vi "VIH HelpGen - Control Label to Control ID.vi"(11 "Control Name":string) -> (3 "Control ID":string)   [LabVIEW 2014]
doc: "::: VI Helpeks :::\nCopyright (c) 2000-2026 Konstantin Shifershteyn. All rights reserved."
panel:
  # "VI Helpeks\nCopyright (c) 2012-2026 Konstantin Shifershteyn"
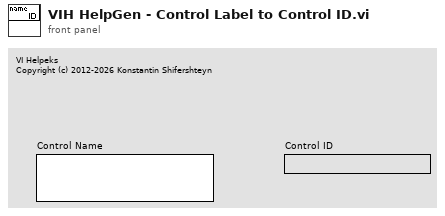
[diagram p1: front panel]
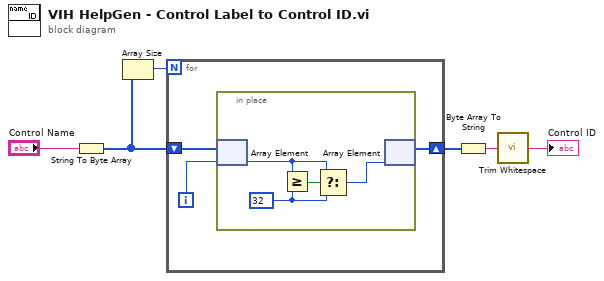
[diagram p0: block diagram]
diagram:
  n1 = String To Byte Array(string="Control Name") -> (unsigned byte array=w1:u8[])
  n2 = Array Size(array=w1) -> (size(s)=w2:i32)
  n3 = for {
    N: w2 -> [_]
    shift-right: [w7] -> w3
    shift-left: w1 -> [w9]
    i -> [w8]
    n4 = in-place {
      w11 = u8 32
      n5 = in-place-array #1(w9, w8) -> (w13:u8)
      n6 = Greater Or Equal?(x=w13, y=w11) -> (x >= y?=w12:bool)
      n7 = Select(t=w13, s=w12, f=w11) -> (s? t:f=w10:u8)
      n8 = in-place-array #1(w10) -> (w7:u8[])  [unwired: 1 out]
    }
  }
  n9 = Byte Array To String(unsigned byte array=w3) -> (string=w5:string)
  n10 = call <vilib>:"Trim Whitespace.vi"("string"=w5) -> ("trimmed string"=→"Control ID":string)  [unwired: 1 in]
